vi "generate default line.vi"(8 "error in":errorcluster, 10 "last line":T1, 11 "Mb Config":refnum<class "Modbus Module configuration.lvclass">) -> (0 "error out":errorcluster, 2 "line":T1, 3 "Modbus Slave configuration out":refnum<class "Modbus Module configuration.lvclass">)   [LabVIEW 2015, in "Modbus Module editor node.lvclass"]
doc: "Platypus Framework 1.0.1.65\nNI Systems Engineering - National Instruments"
uses:
  Modbus Module editor node.lvclass
  table line.ctl
  module/module channel/Modbus Module Channel.lvclass
  module/configuration/Modbus Module configuration.lvclass
  <vilib>/NI/Tag Bus/tag/tag descriptor.lvclass/tag descriptor.ctl
  module/module channel/Modbus Module Channel.lvclass/Modbus Module Channel.ctl
  <vilib>/NI/Tag Bus/tag/Data Type.ctl
  module/module channel/data bank type.ctl
  <vilib>/NI/Tag Bus/tag/read tag name.vi
  <vilib>/NI/Tag Bus/tag/read data type.vi
  module/module channel/Read modbus type.vi
  <vilib>/NI/Tag Bus/tag/write data type.vi
  module/module channel/Write modbus type.vi
  module/module channel/Write starting address.vi
  <vilib>/NI/Tag Bus/tag/write tag name.vi
  <vilib>/NI/Tag Bus/tag/tag descriptor.lvclass
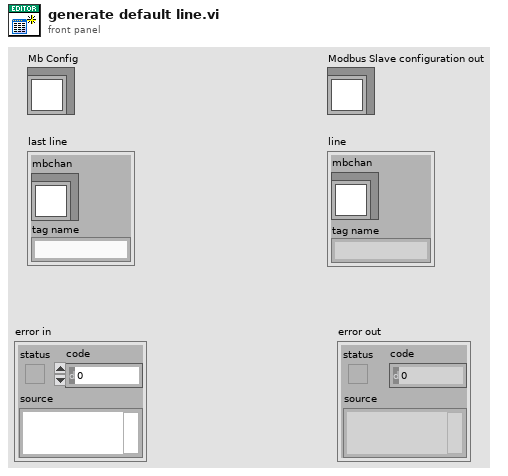
[diagram p1: front panel]
types:
  T1 = typedef "Modbus Module editor node.lvclass/table line.ctl" = cluster{"mbchan":refnum<class "Modbus Module Channel.lvclass">, "tag name":string}
  T2 = typedef "tag bus.lvlib/tag descriptor.lvclass/Data Type.ctl" = enum16{"Double", "Single", "I64", "I32", "I16", "I8", "U64", "U32", "U16", "U8", "Boolean", "String", "Array of Double", "Array of Single", "Array of I64", "Array of I32", "Array of I16", "Array of I8", "Array of U64", "Array of U32", "Array of U16", "Array of U8", "Array of Boolean", "Array of String"}
  T3 = typedef "Modbus Module Channel.lvclass/data bank type.ctl" = enum16{"Coils", "Discrete Inputs", "Input Registers", "Holding Registers"}
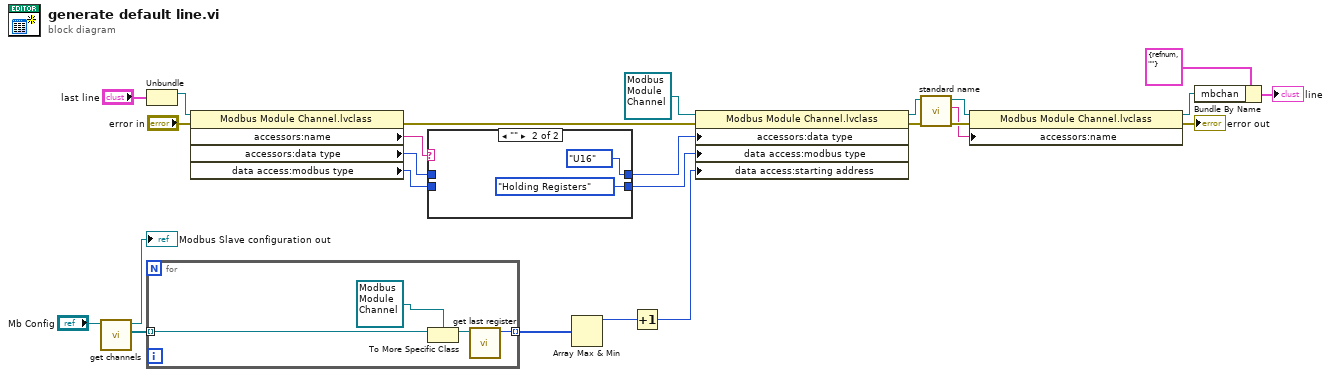
[diagram p0: block diagram]
diagram:
  n1 = call-dynamic "get channels.vi"("Modbus Slave configuration in"="Mb Config") -> ("channels"=w4:refnum<class "TBM channel.lvclass">[], "Modbus Slave configuration out"=→"Modbus Slave configuration out":refnum<class "Modbus Module configuration.lvclass">)  [unwired: 9 in]
  n2 = Unbundle("last line") -> ("mbchan"=w7:refnum<class "Modbus Module Channel.lvclass">)  [unwired: 1 out]
  n3 = for {
    tunnel: [w29] -> w16 mode=indexing
    tunnel: w4 -> [w27] mode=indexing
    n4 = To More Specific Class(target class=refnum<class "Modbus Module Channel.lvclass"> refnum ("Modbus Module Channel in"), reference=w27) -> (specific class reference=w26:refnum<class "Modbus Module Channel.lvclass">)  [unwired: 1 in, 1 out]
    n5 = call "get last register.vi"("Modbus Module Channel in"=w26) -> ("last element"=w29:i32)  [unwired: 10 in]
  }
  n6 = property class="Modbus Module Channel.lvclass"(reference=w7, error in="error in") -> (error out=w1:errorcluster, "accessors:name"=w21:string, "accessors:data type"=w18:T2, "data access:modbus type"=w17:T3)  [unwired: 1 out]
  n7 = case shown="\"\"" w21 {
    tunnel: [w31 Data_Type."U16" ("data type")] -> w20
    tunnel: [w30 data_bank_type."Holding Registers" ("modbus type")] -> w19
    tunnel: w18 -> [w31 _]
    tunnel: w17 -> [w30 _]
    frame Default {
    }
    frame "" {
    }
  }
  n8 = Array Max & Min(array=w16) -> (max value=w15:i32)  [unwired: 3 out]
  n9 = Increment(x=w15) -> (x+1=w14:i32)
  n10 = property class="Modbus Module Channel.lvclass"(reference=refnum<class "Modbus Module Channel.lvclass"> refnum ("Modbus Module Channel"), error in=w1, "accessors:data type"=w20, "data access:modbus type"=w19, "data access:starting address"=w14) -> (reference out=w11:refnum<class "Modbus Module Channel.lvclass">, error out=w10:errorcluster)
  n11 = call "standard name.vi"("error in"=w10, "Modbus Module Channel in"=w11) -> ("error out"=w9:errorcluster, "standard name"=w8:string, "Modbus Module Channel out"=w12:refnum<class "Modbus Module Channel.lvclass">)  [unwired: 7 in]
  n12 = property class="Modbus Module Channel.lvclass"(reference=w12, error in=w9, "accessors:name"=w8) -> (reference out=w13:refnum<class "Modbus Module Channel.lvclass">, error out=→"error out":errorcluster)
  n13 = Bundle By Name(cluster=T1 {"mbchan"=refnum, "tag name"=""} ("line"), "mbchan"=w13) -> (→"line":T1)
